vi "Good Outcome.vi"(10 "stock":i32, 11 "odds":dbl=0.5) -> (3 "good?":bool)   [LabVIEW 2020, in "Full Featured MCP Server.lvlib"]
doc: "Decides whether something turns out well for a stock. odds is the chance for an average company; a strong company (quality 1) gets 25 percentage points more, a weak one (quality -1) as many less."
uses:
  Full Featured MCP Server.lvlib
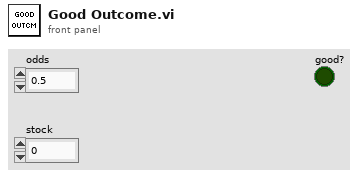
[diagram p1: front panel]
types:
  T1 = cluster{"name":string, "sector":i32, "quality":i32, "start price":dbl, "drift":dbl, "volatility":dbl, "beta":dbl, "jumpiness":dbl, "description":string}[]
  T2 = cluster{"name":string, "sector":i32, "quality":i32, "start price":dbl, "drift":dbl, "volatility":dbl, "beta":dbl, "jumpiness":dbl, "description":string}
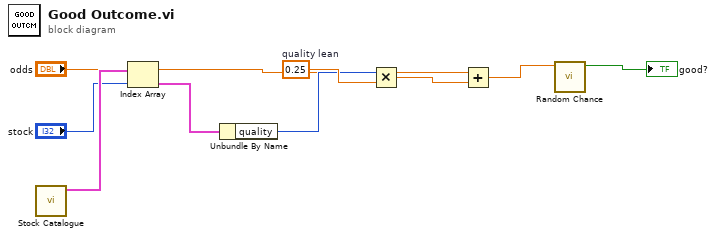
[diagram p0: block diagram]
diagram:
  w6 = 0.25  # quality lean
  n1 = call "Stock Catalogue.vi"() -> ("stocks"=w3:T1)  [unwired: 10 in, 1 out]
  n2 = Index Array(array=w3, index="stock") -> (element=w4:T2)
  n3 = Unbundle By Name(w4) -> ("quality"=w5:i32)
  n4 = Multiply(x=w5, y=w6) -> (x*y=w7:dbl)
  n5 = Add(x="odds", y=w7) -> (x+y=w8:dbl)
  n6 = call "Random Chance.vi"("probability"=w8) -> ("happened?"=→"good?":bool)  [unwired: 10 in]
